vi "lab1_FPGA.vi"() -> ()   [LabVIEW 2025]
uses:
  <vilib>/Platform/TimedLoop/XDataNode/timing_clust.ctl
  <vilib>/Platform/TimedLoop/XDataNode/nitl_modes.ctl
  <vilib>/Platform/TimedLoop/XDataNode/wakeup.ctl
  <vilib>/rvi/Emulation/niFpgaGetClockAttributes.vi
  <vilib>/rvi/Emulation/niFpgaSctlEmulationGetInTimedLoop.vi
  <vilib>/rvi/Emulation/niFpgaEmulationReportErrorSimple.vi
  <vilib>/rvi/eio/common/nirviEmuTemplateMethod_errors.vi
  <vilib>/rvi/Emulation/niFpgaCriticalErrorInLSC.vi
  <vilib>/eio/EIONode/EIONode.xnode
  <vilib>/platform/TimedLoop/XDataNode/XDataNode.xnode
  <vilib>/Platform/TimedLoop/XDataNode/XDNodeRunTimeDep.lvlib
panel:
  in  "Period":i64
  in  "Count(Ticks)":u32 caption="Count(us)"
  in  "N":i16
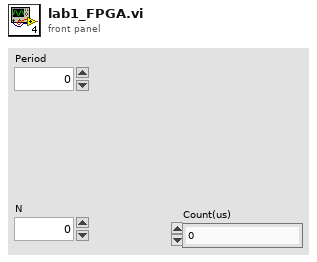
[diagram p1: front panel]
types:
  T1 = typedef "XDNodeRunTimeDep.lvlib/timing_clust.ctl" = cluster{"Expected End [f-1]":u64, "Actual End [f-1]":u64, "Finished Late? [f-1]":bool, "Expected End [i-1]":u64, "Actual End [i-1]":u64, "Finished Late? [i-1]":bool, "Expected Start [i]":u64, "Actual Start [i]":u64, "Expected Start [f]":u64, "Actual Start [f]":u64, "Source Name":string, "Structure Name":string, "Period":i64, "Deadline":i64, "Offset":i64, "Start":i64, "Priority":i32, "Timeout":i32, "Mode":T2, "Wakeup Reason":T3, "Error":errorcluster, "Source Type":string, "Secondary Source Type":string, "Global End Time":u64, "Global Start Time":u64, "Frame Duration":u64, "Iteration Duration":u64, "Assigned CPU":i32, "I/O Scan Engine Mode":u32}
  T2 = typedef "XDNodeRunTimeDep.lvlib/nitl_modes.ctl" = enum32{"No Change", "Process missed periods, maintain original phase", "Discard missed periods, maintain original phase", "Process missed periods, ignore original phase", "Discard missed periods, ignore original phase"}
  T3 = typedef "XDNodeRunTimeDep.lvlib/wakeup.ctl" = enum32{"Normal", "Aborted", "Asynchronous wakeup", "Timing source error", "Timed loop error", "Timeout"}
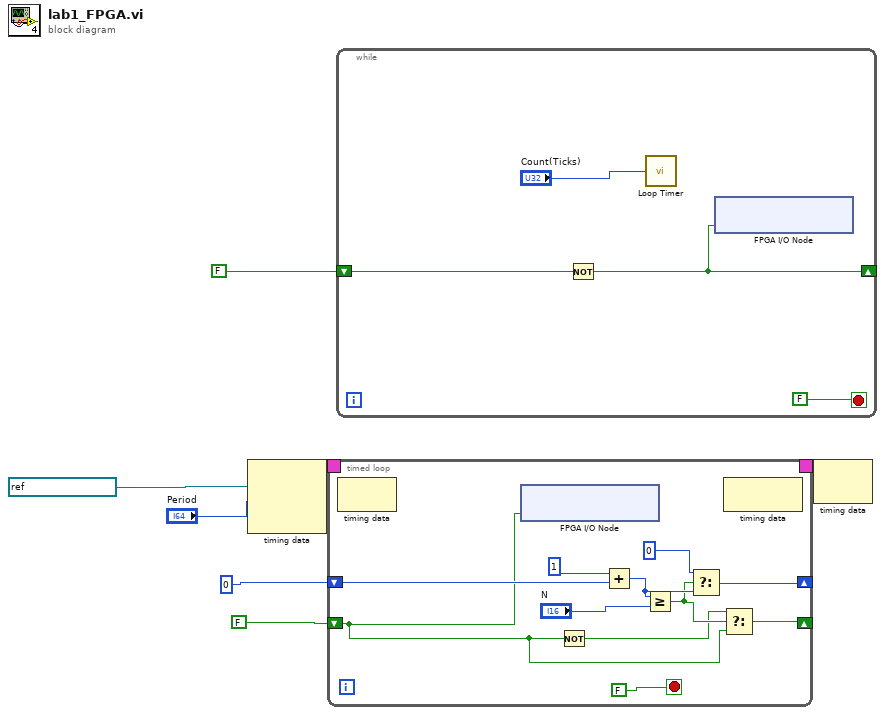
[diagram p0: block diagram]
diagram:
  n1 = node-c288(refnum<k21> "40 MHz Onboard Clock" ("Source Name"), "Period") -> (w7:T1)  [unwired: 1 in]
  n2 = timed-loop {
    timing: w7 -> [_]
    timing-out: [_] -> w6
    shift-right: [w9] -> _
    shift-left: FALSE -> [w8]
    shift-right: [w12] -> _
    shift-left: i16 0 -> [w17]
    stop <- FALSE stop-if-true
    n3 = node-c288() -> ()  [unwired: 1 in, 1 out]
    n4 = xnode "FPGA I/O Node"("ConnectorA/DIO2"=w8) -> ()  [unwired: 1 in, 1 out]
    n5 = Not(x=w8) -> (.not. x?=w10:bool)
    n6 = Add(x=i16 1, y=w17) -> (x+y=w14:i16)
    n7 = Greater Or Equal?(x=w14, y="N") -> (x >= y?=w11:bool)
    n8 = Select(t=i16 0, s=w11, f=w14) -> (s? t:f=w12:i16)
    n9 = node-c288() -> ()  [unwired: 1 in, 1 out]
    n10 = Select(t=w10, s=w11, f=w8) -> (s? t:f=w9:bool)
  }
  n11 = while {
    shift-right: [w22] -> _
    shift-left: FALSE -> [w24]
    stop <- FALSE stop-if-true
    n12 = Not(x=w24) -> (.not. x?=w22:bool)
    n13 = call "Loop Timer"("Count(uSec)"="Count(Ticks)") -> ()  [unwired: 1 out]
    n14 = xnode "FPGA I/O Node"("ConnectorA/DIO1"=w22) -> ()  [unwired: 1 in, 1 out]
  }
  n15 = node-c288(w6) -> ()  [unwired: 1 out]
